vi "Control - Spark.vi"(8 "Control Inputs":T1={"Engine Speed [RPM]"=0.0, "Engine Status"=enum."STALLED", "Load Control \nMode"=enum."Max Speed Governor", "dt(s)"=0.0, "Number of Cylinders"=0, "Engine Displacement [cc]"=0.0, "StoichAFR"=0.0, "Q.LHV Fuel [kJ/kg]"=0.0, "BattV PSU [V]"=0.0, "12V PSU [V]"=0.0, "5V PSU [V]"=0.0, "Pedal Position [%]"=0.0, "Oil Pressure [kPa]"=0.0, "Oil Temp [C]"=0.0, "Oil Level [%]"=0.0, "Engine Coolant Temp (ECT) [C]"=0.0, "Engine Coolant Pressure [kPa]"=0.0, "Rail Pressure [bar]"=0.0, "Fuel Pressure [kPa]"=0.0, "Fuel Temp [C]"=0.0, "Vacuum Pressure [kPa]"=0.0, "Throttle Position [%]"=0.0, "Cam1 Advance [CAD]"=0.0, "Cam2 Advance [CAD]"=0.0, "Cam3 Advance [CAD]"=0.0, "Cam4 Advance [CAD]"=0.0, "CA50 Control Output [CAD]"=[], "CA50 Control Output Valid"=[], "Intake Air Temp (IAT) [C]"=0.0, "Barometric Air Pressure [kPa]"=0.0, "Intake Air Rel. Humidity [%]"=0.0, "Mass Air Flow (MAF) [kg/hr]"=0.0, "Turbo Inlet Air Pressure [kPa]"=0.0, "Turbo Inlet Air Temp [C]"=0.0, "Turbo Outlet Air Pressure [kPa]"=0.0, "Turbo Outlet Air Temp [C]"=0.0, "CAC Outlet Pressure [kPa]"=0.0, "CAC Outlet Temp [C]"=0.0, "Intake Manifold Pressure (MAP) [kPa]"=0.0, "Intake Manifold Temp (MAT) [C]"=0.0, "Exhaust Manifold Pressure [kPa]"=0.0, "Exhaust Manifold Temp [C]"=0.0, "HighP EGR Cooler Outlet Pressure [kPa]"=0.0, "HighP EGR Cooler Outlet Temp [C]"=0.0, "HighP EGR Differential Pressure [kPa]"=0.0, "HighP EGR Valve Position [%]"=0.0, "Turbo Outlet Exhaust Pressure [kPa]"=0.0, "Turbo Outlet Exhaust Temp [C]"=0.0, "VGT Position 1 [%]"=0.0, "VGT Position 2 [%]"=0.0, "Turbo Speed 1 [RPM]"=0.0, "Turbo Speed 2 [RPM]"=0.0, "LowP EGR Differential Pressure [kPa]"=0.0, "LowP EGR Valve Position [%]"=0.0, "UEGO1Lambda"=0.0, "UEGO1_Hot"=FALSE, "UEGO2Lambda"=0.0, "UEGO2_Hot"=FALSE, "Knock Intensity"=[], "Knock"=[]} {"Knock Intensity" format="%.2f"; "CA50 Control Output [CAD]" format="%.2f"; "Exhaust Manifold Temp [C]" format="%#_6f"; "UEGO2Lambda" format="%.2f"; "Intake Manifold Temp (MAT) [C]" format="%#_6f"; "UEGO1Lambda" format="%.2f"}, 10 "EGR Mass [mg/cyc]":sgl, 11 "MEP Desired [bar]":sgl) -> (1 "Spark Timings Desired [DBTDC]":sgl[](array[numeric]), 3 "Spark Dwells Desired [msec]":sgl[](array[numeric]))   [LabVIEW 2015, in "ECS-RT.lvlib"]
uses:
  ECS-RT.lvlib
  Typedefs/Control Inputs/Control Inputs.ctl
  Typedefs/EPT/Engine Status.ctl
  Typedefs/MISC/Load Control Mode.ctl
  ECS-Shared.lvlib
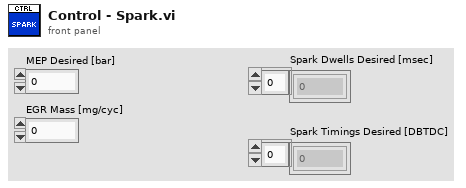
[diagram p1: front panel]
types:
  T1 = typedef "ECS-Shared.lvlib/Control Inputs.ctl" = cluster{"Engine Speed [RPM]":sgl, "Engine Status":T2, "Load Control \nMode":T3, "dt(s)":sgl, "Number of Cylinders":u8, "Engine Displacement [cc]":sgl, "StoichAFR":sgl, "Q.LHV Fuel [kJ/kg]":sgl, "BattV PSU [V]":sgl, "12V PSU [V]":sgl, "5V PSU [V]":sgl, "Pedal Position [%]":sgl, "Oil Pressure [kPa]":sgl, "Oil Temp [C]":sgl, "Oil Level [%]":sgl, "Engine Coolant Temp (ECT) [C]":sgl, "Engine Coolant Pressure [kPa]":sgl, "Rail Pressure [bar]":sgl, "Fuel Pressure [kPa]":sgl, "Fuel Temp [C]":sgl, "Vacuum Pressure [kPa]":sgl, "Throttle Position [%]":sgl, "Cam1 Advance [CAD]":sgl, "Cam2 Advance [CAD]":sgl, "Cam3 Advance [CAD]":sgl, "Cam4 Advance [CAD]":sgl, "CA50 Control Output [CAD]":sgl[], "CA50 Control Output Valid":bool[], "Intake Air Temp (IAT) [C]":sgl, "Barometric Air Pressure [kPa]":sgl, "Intake Air Rel. Humidity [%]":sgl, "Mass Air Flow (MAF) [kg/hr]":sgl, "Turbo Inlet Air Pressure [kPa]":sgl, "Turbo Inlet Air Temp [C]":sgl, "Turbo Outlet Air Pressure [kPa]":sgl, "Turbo Outlet Air Temp [C]":sgl, "CAC Outlet Pressure [kPa]":sgl, "CAC Outlet Temp [C]":sgl, "Intake Manifold Pressure (MAP) [kPa]":sgl, "Intake Manifold Temp (MAT) [C]":sgl, "Exhaust Manifold Pressure [kPa]":sgl, "Exhaust Manifold Temp [C]":sgl, "HighP EGR Cooler Outlet Pressure [kPa]":sgl, "HighP EGR Cooler Outlet Temp [C]":sgl, "HighP EGR Differential Pressure [kPa]":sgl, "HighP EGR Valve Position [%]":sgl, "Turbo Outlet Exhaust Pressure [kPa]":sgl, "Turbo Outlet Exhaust Temp [C]":sgl, "VGT Position 1 [%]":sgl, "VGT Position 2 [%]":sgl, "Turbo Speed 1 [RPM]":sgl, "Turbo Speed 2 [RPM]":sgl, "LowP EGR Differential Pressure [kPa]":sgl, "LowP EGR Valve Position [%]":sgl, "UEGO1Lambda":sgl, "UEGO1_Hot":bool, "UEGO2Lambda":sgl, "UEGO2_Hot":bool, "Knock Intensity":sgl[], "Knock":bool[]}
  T2 = typedef "ECS-Shared.lvlib/Engine Status.ctl" = enum16{"OFF", "STALLED", "CRANKING", "RUNNING", "ACCEL", "DECEL", "SAFE"}
  T3 = typedef "ECS-Shared.lvlib/Load Control Mode.ctl" = enum16{"No Governor", "Min Speed Governor", "Max Speed Governor"}
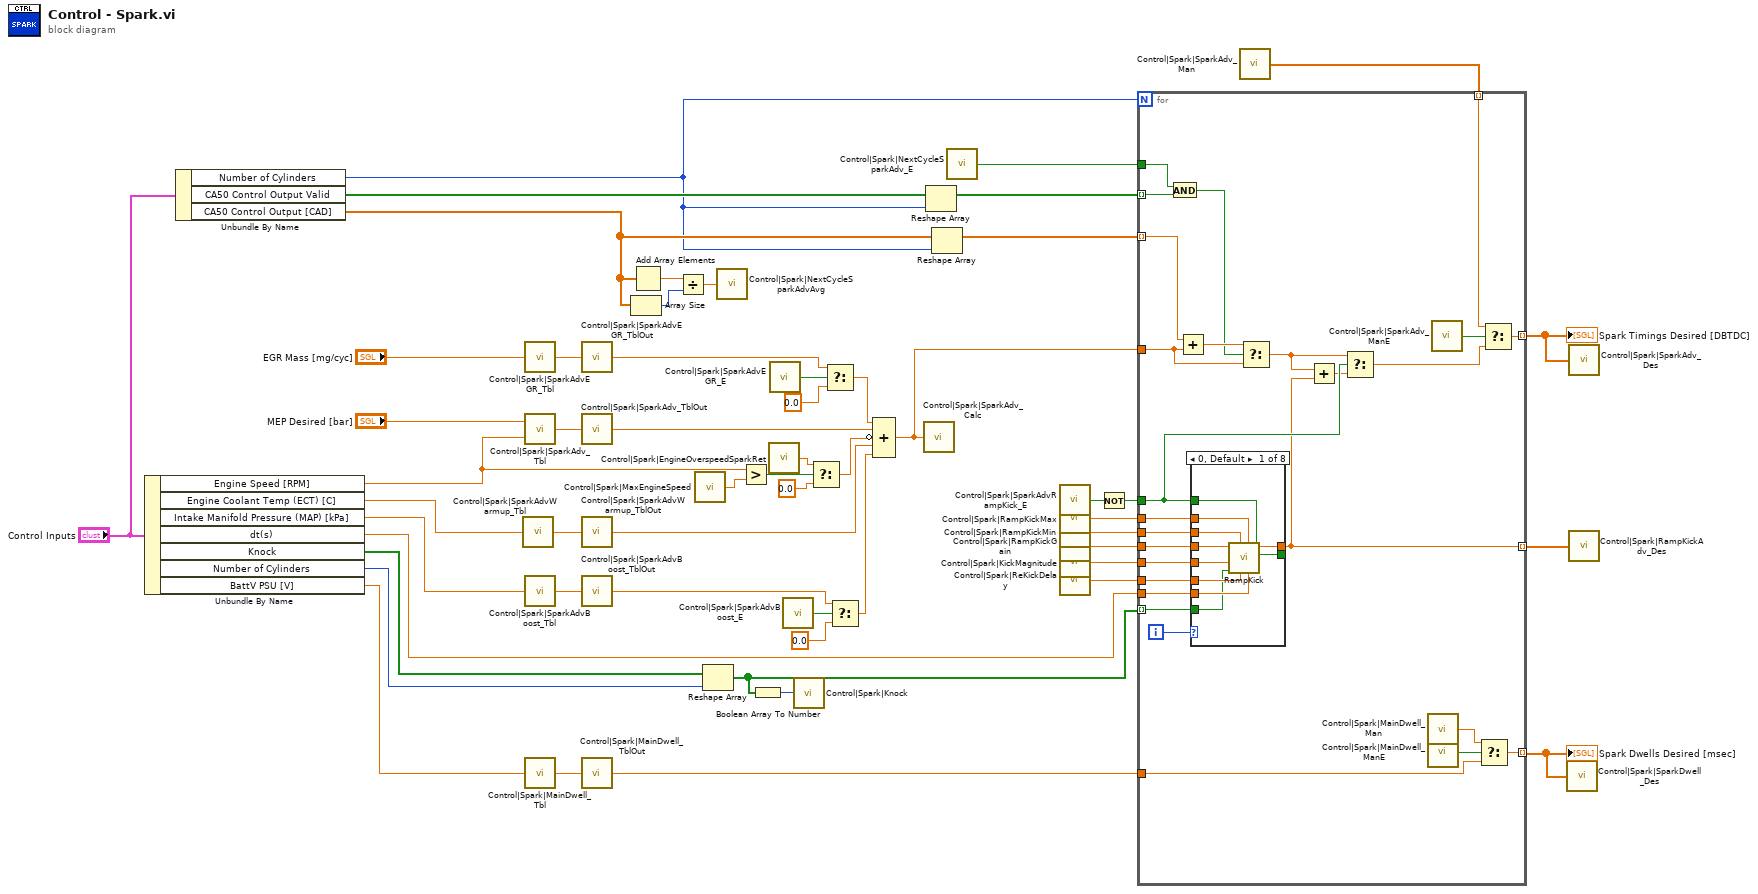
[diagram p0: block diagram]
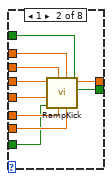
[diagram p2: hidden frame]
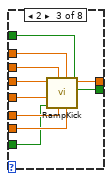
[diagram p3: hidden frame]
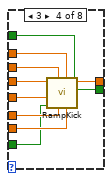
[diagram p4: hidden frame]
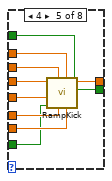
[diagram p5: hidden frame]
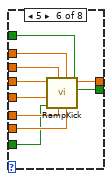
[diagram p6: hidden frame]
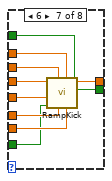
[diagram p7: hidden frame]
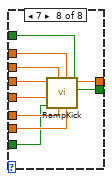
[diagram p8: hidden frame]
diagram:
  n1 = Unbundle By Name("Control Inputs") -> ("Engine Speed [RPM]"=w27:sgl, "Engine Coolant Temp (ECT) [C]"=w22:sgl, "Intake Manifold Pressure (MAP) [kPa]"=w23:sgl, "dt(s)"=w12:sgl, "Knock"=w3:bool[], "Number of Cylinders"=w1:u8, "BattV PSU [V]"=w15:sgl)
  n2 = Unbundle By Name("Control Inputs") -> ("Number of Cylinders"=w4:u8, "CA50 Control Output Valid"=w6:bool[], "CA50 Control Output [CAD]"=w8:sgl[])
  n3 = call "Control|Spark|SparkAdvWarmup_Tbl"("X Index"=w22) -> ("Y"=w30:sgl)
  n4 = call "Control|Spark|SparkAdvEGR_Tbl"("X Index"="EGR Mass [mg/cyc]") -> ("Y"=w35:sgl)
  n5 = call "Control|Spark|SparkAdv_Tbl"("Y Index"=w27, "X Index"="MEP Desired [bar]") -> ("Z"=w36:sgl)
  n6 = call "Control|Spark|SparkAdvBoost_Tbl"("X Index"=w23) -> ("Y"=w37:sgl)
  n7 = call "Control|Spark|MainDwell_Tbl"("X Index"=w15) -> ("Y"=w38:sgl)
  n8 = call "Control|Spark|SparkAdvEGR_TblOut"("Value"=w35) -> ()
  n9 = call "Control|Spark|SparkAdv_TblOut"("Value"=w36) -> ()
  n10 = call "Control|Spark|SparkAdvWarmup_TblOut"("Value"=w30) -> ()
  n11 = call "Control|Spark|SparkAdvBoost_TblOut"("Value"=w37) -> ()
  n12 = call "Control|Spark|MainDwell_TblOut"("Value"=w38) -> ()
  n13 = Array Size(array=w8) -> (size(s)=w41:i32)
  n14 = Add Array Elements(numeric array=w8) -> (sum=w42:sgl)
  n15 = Divide(x=w42, y=w41) -> (x/y=w40:sgl)
  n16 = call "Control|Spark|MaxEngineSpeed"() -> ("Value"=w21:sgl)
  n17 = Reshape Array(w3, w1) -> (w2:bool[])
  n18 = call "Control|Spark|NextCycleSparkAdvAvg"("Value"=w40) -> ()
  n19 = Greater?(x=w27, y=w21) -> (0:w29:bool)
  n20 = Boolean Array To Number(Boolean array=w2) -> (number=w14:u8)
  n21 = call "Control|Spark|EngineOverspeedSparkRet"() -> ("Value"=w26:sgl)
  n22 = call "Control|Spark|SparkAdvEGR_E"() -> ("Value"=w46:bool)
  n23 = call "Control|Spark|SparkAdvBoost_E"() -> ("Value"=w47:bool)
  n24 = call "Control|Spark|Knock"("Value"=w14) -> ()
  n25 = Select(t=w26, s=w29, f=sgl 0.0) -> (s? t:f=w28:sgl)
  n26 = Select(t=w35, s=w46, f=sgl 0.0) -> (s? t:f=w43:sgl)
  n27 = Select(t=w37, s=w47, f=sgl 0.0) -> (s? t:f=w31:sgl)
  n28 = Compound Arithmetic op=ADD(w43, w36, invert w28, w30, w31) -> (w32:sgl)
  n29 = call "Control|Spark|SparkAdv_Calc"("Value"=w32) -> ()
  n30 = Reshape Array(w6, w4) -> (w5:bool[])
  n31 = Reshape Array(w8, w4) -> (w7:sgl[])
  n32 = call "Control|Spark|NextCycleSparkAdv_E"() -> ("Value"=w39:bool)
  n33 = call "Control|Spark|SparkAdvRampKick_E"() -> ("Value"=w13:bool)
  n34 = call "Control|Spark|RampKickMax"() -> ("Value"=w20:sgl)
  n35 = call "Control|Spark|RampKickMin"() -> ("Value"=w19:sgl)
  n36 = call "Control|Spark|RampKickGain"() -> ("Value"=w18:sgl)
  n37 = call "Control|Spark|KickMagnitude"() -> ("Value"=w17:sgl)
  n38 = call "Control|Spark|ReKickDelay"() -> ("Value"=w16:sgl)
  n39 = Not(x=w13) -> (.not. x?=w11:bool)
  n40 = call "Control|Spark|SparkAdv_Man"() -> ("Value"=w9:sgl[])
  n41 = for {
    N: w4 -> [_]
    tunnel: w32 -> [w69]
    tunnel: w38 -> [w73]
    tunnel: [w72] -> w33 mode=indexing
    tunnel: [w71] -> w34 mode=indexing
    tunnel: w5 -> [w50] mode=indexing
    tunnel: w7 -> [w68] mode=indexing
    tunnel: w39 -> [w51]
    tunnel: w20 -> [w64]
    tunnel: w19 -> [w63]
    tunnel: w18 -> [w62]
    tunnel: w17 -> [w61]
    tunnel: w16 -> [w60]
    tunnel: w12 -> [w59]
    tunnel: w2 -> [w58] mode=indexing
    tunnel: w11 -> [w56]
    tunnel: [w53] -> w10 mode=indexing
    tunnel: w9 -> [w52] mode=indexing
    i -> [w65]
    n42 = And(x=w51, y=w50) -> (x .and. y?=w66:bool)
    n43 = Add(x=w68, y=w69) -> (x+y=w70:sgl)
    n44 = case shown="0, Default" w65 {
      tunnel: w63 -> [w85 w95 w105 w115 w125 w135 w145 w155]
      tunnel: w64 -> [w84 w94 w104 w114 w124 w134 w144 w154]
      tunnel: w62 -> [w83 w93 w103 w113 w123 w133 w143 w153]
      tunnel: w61 -> [w82 w92 w102 w112 w122 w132 w142 w152]
      tunnel: w60 -> [w81 w91 w101 w111 w121 w131 w141 w151]
      tunnel: w59 -> [w80 w90 w100 w110 w120 w130 w140 w150]
      tunnel: w58 -> [w79 w89 w99 w109 w119 w129 w139 w149]
      tunnel: [w78 w88 w98 w108 w118 w128 w138 w148] -> w53
      tunnel: [w77 w87 w97 w107 w117 w127 w137 w147] -> _
      tunnel: w56 -> [w76 w86 w96 w106 w116 w126 w136 w146]
      frame 0, Default {
        n45 = call "RampKick.vi"("Init (F)"=w76, "dt [s]"=w80, "Output Max [unit]"=w84, "Re-Kick Delay [s]"=w81, "Output Min [unit]"=w85, "Kick?"=w79, "Kick Magnitude [unit]"=w82, "Gain [unit/s]"=w83) -> ("Kicked"=w77:bool, "Ramp/Kick Output"=w78:sgl)  [unwired: 2 in]
      }
      frame 1 {
        n46 = call "RampKick.vi"("Init (F)"=w86, "dt [s]"=w90, "Output Max [unit]"=w94, "Re-Kick Delay [s]"=w91, "Output Min [unit]"=w95, "Kick?"=w89, "Kick Magnitude [unit]"=w92, "Gain [unit/s]"=w93) -> ("Kicked"=w87:bool, "Ramp/Kick Output"=w88:sgl)  [unwired: 2 in]
      }
      frame 2 {
        n47 = call "RampKick.vi"("Init (F)"=w96, "dt [s]"=w100, "Output Max [unit]"=w104, "Re-Kick Delay [s]"=w101, "Output Min [unit]"=w105, "Kick?"=w99, "Kick Magnitude [unit]"=w102, "Gain [unit/s]"=w103) -> ("Kicked"=w97:bool, "Ramp/Kick Output"=w98:sgl)  [unwired: 2 in]
      }
      frame 3 {
        n48 = call "RampKick.vi"("Init (F)"=w106, "dt [s]"=w110, "Output Max [unit]"=w114, "Re-Kick Delay [s]"=w111, "Output Min [unit]"=w115, "Kick?"=w109, "Kick Magnitude [unit]"=w112, "Gain [unit/s]"=w113) -> ("Kicked"=w107:bool, "Ramp/Kick Output"=w108:sgl)  [unwired: 2 in]
      }
      frame 4 {
        n49 = call "RampKick.vi"("Init (F)"=w116, "dt [s]"=w120, "Output Max [unit]"=w124, "Re-Kick Delay [s]"=w121, "Output Min [unit]"=w125, "Kick?"=w119, "Kick Magnitude [unit]"=w122, "Gain [unit/s]"=w123) -> ("Kicked"=w117:bool, "Ramp/Kick Output"=w118:sgl)  [unwired: 2 in]
      }
      frame 5 {
        n50 = call "RampKick.vi"("Init (F)"=w126, "dt [s]"=w130, "Output Max [unit]"=w134, "Re-Kick Delay [s]"=w131, "Output Min [unit]"=w135, "Kick?"=w129, "Kick Magnitude [unit]"=w132, "Gain [unit/s]"=w133) -> ("Kicked"=w127:bool, "Ramp/Kick Output"=w128:sgl)  [unwired: 2 in]
      }
      frame 6 {
        n51 = call "RampKick.vi"("Init (F)"=w136, "dt [s]"=w140, "Output Max [unit]"=w144, "Re-Kick Delay [s]"=w141, "Output Min [unit]"=w145, "Kick?"=w139, "Kick Magnitude [unit]"=w142, "Gain [unit/s]"=w143) -> ("Kicked"=w137:bool, "Ramp/Kick Output"=w138:sgl)  [unwired: 2 in]
      }
      frame 7 {
        n52 = call "RampKick.vi"("Init (F)"=w146, "dt [s]"=w150, "Output Max [unit]"=w154, "Re-Kick Delay [s]"=w151, "Output Min [unit]"=w155, "Kick?"=w149, "Kick Magnitude [unit]"=w152, "Gain [unit/s]"=w153) -> ("Kicked"=w147:bool, "Ramp/Kick Output"=w148:sgl)  [unwired: 2 in]
      }
    }
    n53 = Select(t=w70, s=w66, f=w69) -> (s? t:f=w54:sgl)
    n54 = Add(x=w54, y=w53) -> (x+y=w55:sgl)
    n55 = Select(t=w54, s=w56, f=w55) -> (s? t:f=w57:sgl)
    n56 = call "Control|Spark|MainDwell_Man"() -> ("Value"=w67:sgl)
    n57 = call "Control|Spark|MainDwell_ManE"() -> ("Value"=w74:bool)
    n58 = call "Control|Spark|SparkAdv_ManE"() -> ("Value"=w75:bool)
    n59 = Select(t=w67, s=w74, f=w73) -> (s? t:f=w72:sgl)
    n60 = Select(t=w52, s=w75, f=w57) -> (s? t:f=w71:sgl)
  }
  "Spark Timings Desired [DBTDC]" <- w34
  "Spark Dwells Desired [msec]" <- w33
  n61 = call "Control|Spark|SparkDwell_Des"("Value"=w33) -> ()
  n62 = call "Control|Spark|SparkAdv_Des"("Value"=w34) -> ()
  n63 = call "Control|Spark|RampKickAdv_Des"("Value"=w10) -> ()
